vi "Read_MemBank.vi"(8 "error in":errorcluster, 10 "Device":T1, 11 "NNPC_Paths":T2) -> (0 "error out":errorcluster, 3 "NNPC_MemBank_and_Params":T3 {"PreProc_Options"."Dataset_Stats"."stds"."R" format="%#_3g"; "PreProc_Options"."Dataset_Stats"."stds"."G" format="%#_3g"; "PreProc_Options"."Dataset_Stats"."stds"."B" format="%#_3g"; "PreProc_Options"."Dataset_Stats"."means"."R" format="%#_3g"; "PreProc_Options"."Dataset_Stats"."means"."G" format="%#_3g"; "PreProc_Options"."Dataset_Stats"."means"."B" format="%#_3g"; "PreProc_Options"."Interpolation Type" items=["Zero Order", "Bi-Linear", "Quadratic", "Cubic Spline"]; "Evaluation_Results"."Pixel_Range"."Min" format="%#_5g"})   [LabVIEW 2020]
uses:
  Controls/NNPC_MemBank_and_Params.ctl
  <vilib>/Ngene/DeepLTK Anomaly Detection Addon/Toolkit/API/Controls/MemBank_and_Norm_Variants.ctl
  <vilib>/Ngene/DeepLTK Anomaly Detection Addon/Toolkit/API/Controls/NNPC_PreProcessing_Options.ctl
  <vilib>/Ngene/Deep Learning Toolkit/Toolkit/NN_Data/API/NN_Dims(C,H,W).ctl
  <vilib>/Ngene/DeepLTK Anomaly Detection Addon/Toolkit/API/Controls/Crop_CFG.ctl
  <vilib>/Ngene/DeepLTK Anomaly Detection Addon/Toolkit/API/Controls/NNPC_DS_Stats.ctl
  <vilib>/Ngene/DeepLTK Anomaly Detection Addon/Toolkit/API/Controls/Image_Stats_RGB.ctl
  <vilib>/Ngene/DeepLTK Anomaly Detection Addon/Toolkit/API/Controls/NNPC_Evaluation_Results.ctl
  <vilib>/Ngene/DeepLTK Anomaly Detection Addon/Toolkit/API/Controls/NN_Paths.ctl
  <vilib>/Ngene/Deep Learning Toolkit/Toolkit/NN_Network/Controls/NN_Device.ctl
  <vilib>/Ngene/DeepLTK Anomaly Detection Addon/Toolkit/API/Controls/NNPC_Setup.ctl
  <vilib>/Ngene/Deep Learning Toolkit/Toolkit/NN_Network/Controls/NN_Save_Before_Destroy_Options.ctl
  <vilib>/Ngene/CuLab - GPU Accelerated Toolkit/Toolkit/Low_Level/Tensor_Classes/T_Children/T2D/T2D_Children/T2D_SGL/Create_Push.vi
  <vilib>/Ngene/CuLab - GPU Accelerated Toolkit/Toolkit/Low_Level/Tensor_Classes/T_Children/T1D/T1D_Children/T1D_SGL/Create_Push.vi
  <vilib>/Ngene/DeepLTK Anomaly Detection Addon/Toolkit/DeepLTK_Anomaly_Detection_Addon.lvlib
  <vilib>/Ngene/Deep Learning Toolkit/Toolkit/Deep_Learning_Toolkit_by_Ngene.lvlib
  <vilib>/Ngene/CuLab - GPU Accelerated Toolkit/Toolkit/CuLab.lvlib
  <vilib>/Ngene/CuLab - GPU Accelerated Toolkit/Toolkit/Low_Level/Tensor_Classes/T_Children/T1D/T1D_Children/T1D_SGL/T1D_SGL.lvclass
  <vilib>/Ngene/CuLab - GPU Accelerated Toolkit/Toolkit/Low_Level/Tensor_Classes/T_Children/T2D/T2D_Children/T2D_SGL/T2D_SGL.lvclass
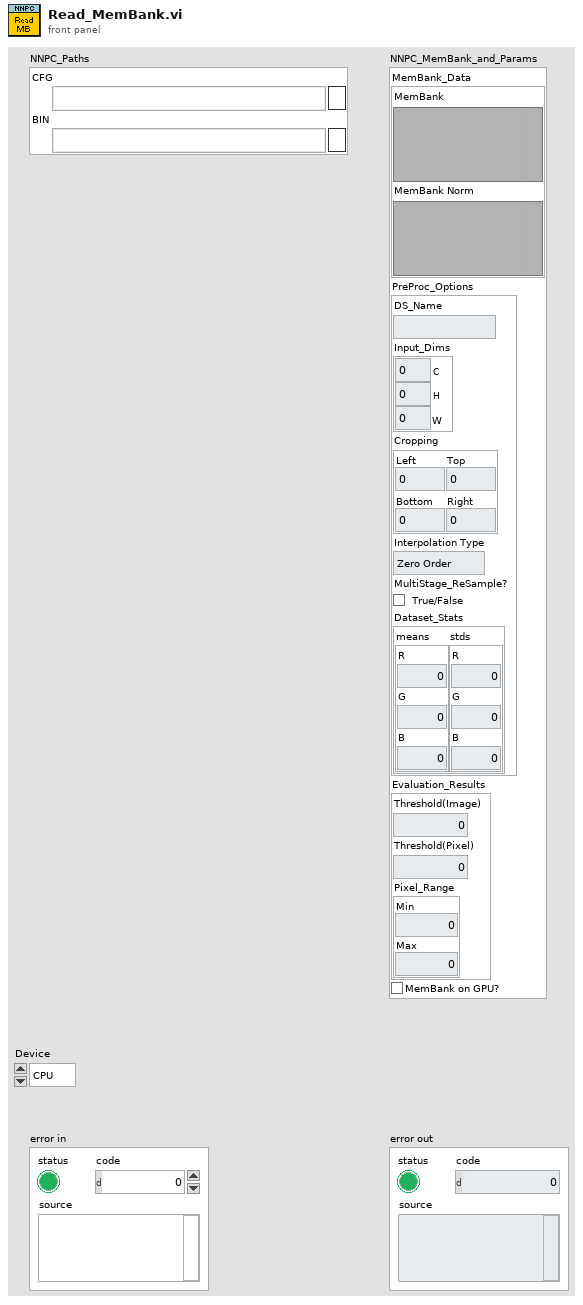
[diagram p1: front panel]
types:
  T1 = typedef "Deep_Learning_Toolkit_by_Ngene.lvlib/NN_Device.ctl" = enum16{"CPU", "GPU"}
  T2 = typedef "DeepLTK_Anomaly_Detection_Addon.lvlib/NN_Paths.ctl" = cluster{"CFG":path, "BIN":path}
  T3 = typedef "NNPC_MemBank_and_Params.ctl" = cluster{"MemBank_Data":T4, "PreProc_Options":T5, "Evaluation_Results":T10, "MemBank on GPU?":bool}
  T4 = typedef "DeepLTK_Anomaly_Detection_Addon.lvlib/MemBank_and_Norm_Variants.ctl" = cluster{"MemBank":variant, "MemBank Norm":variant}
  T5 = typedef "DeepLTK_Anomaly_Detection_Addon.lvlib/NNPC_PreProcessing_Options.ctl" = cluster{"DS_Name":string, "Input_Dims":T6, "Cropping":T7, "Interpolation Type":u32, "MultiStage_ReSample?":bool, "Dataset_Stats":T8}
  T6 = typedef "Deep_Learning_Toolkit_by_Ngene.lvlib/NN_Dims(C,H,W).ctl" = cluster{"C":i32, "H":i32, "W":i32}
  T7 = typedef "DeepLTK_Anomaly_Detection_Addon.lvlib/Crop_CFG.ctl" = cluster{"Left":sgl, "Top":sgl, "Right":sgl, "Bottom":sgl}
  T8 = typedef "DeepLTK_Anomaly_Detection_Addon.lvlib/NNPC_DS_Stats.ctl" = cluster{"means":T9, "stds":T9}
  T9 = typedef "DeepLTK_Anomaly_Detection_Addon.lvlib/Image_Stats_RGB.ctl" = cluster{"R":sgl, "G":sgl, "B":sgl}
  T10 = typedef "DeepLTK_Anomaly_Detection_Addon.lvlib/NNPC_Evaluation_Results.ctl" = cluster{"Threshold(Image)":sgl, "Threshold(Pixel)":sgl, "Pixel_Range":cluster{"Min":sgl, "Max":sgl}}
  T11 = typedef "DeepLTK_Anomaly_Detection_Addon.lvlib/NNPC_Setup.ctl" = cluster{"Input_Dims":T6, "mBatch":i32, "Device":T1, "GPU Id":i32}
  T12 = typedef "Deep_Learning_Toolkit_by_Ngene.lvlib/NN_Save_Before_Destroy_Options.ctl" = cluster{"CFG?":bool, "Weights?":bool, "Render?":bool}
  T13 = typedef "DeepLTK_Anomaly_Detection_Addon.lvlib/NNPC_Instance.ctl" = cluster{"Name":string, "NN":T14, "MemBank_Data":T4}
  T14 = typedef "Deep_Learning_Toolkit_by_Ngene.lvlib/NN.ctl" = cluster{"Name":string, "No of Layers":i32, "mBatch":i32, "Layers":T15[], "Dimty":T16, "Dims_In":T6, "Dims_Out":T6, "Working_Dir":path, "Train?":bool, "Train_Params":T17, "LR_Update_Policy":T20, "Session Data":T22, "Ground_truth":T23, "NNg_hdls":T24, "NN_Device":T1, "GPU Id":i32, "Labels":string[], "Loss_Type":T25, "Loss_Cfg_Prms":variant, "NNG_WS":T26, "DryRun?":bool}
  T15 = typedef "Deep_Learning_Toolkit_by_Ngene.lvlib/NN_Layer_ref.ctl" = refnum<file>
  T16 = typedef "Deep_Learning_Toolkit_by_Ngene.lvlib/NN_In_Out_Dim-ty.ctl" = enum8{"In1D_Out1D", "In3D_Out1D", "In3D_Out3D", "In3D_OutBBox"}
  T17 = typedef "Deep_Learning_Toolkit_by_Ngene.lvlib/NN_Train_Params.ctl" = cluster{"Optimizer":T18, "Beta_1":sgl, "Beta_2":sgl, "Weight Decay(L1)":sgl, "Weight Decay(L2)":sgl, "Data_Sampling":T19}
  T18 = typedef "Deep_Learning_Toolkit_by_Ngene.lvlib/NN_Train_Optimizer.ctl" = enum16{"SGD", "Adam", "Adagrad", "Adadelta", "RMSProp", "Nesterov"}
  T19 = typedef "Deep_Learning_Toolkit_by_Ngene.lvlib/NN_Train_Data_Sampling.ctl" = enum16{"Random", "Sequential"}
  T20 = typedef "Deep_Learning_Toolkit_by_Ngene.lvlib/NN_LR_Policy_Cfg.ctl" = cluster{"Policy_Type":T21, "LR0":dbl, "k":sgl, "WarmUp_Policy":enum16{"Step", "Ramp"}, "WarmUp_Iter":i32, "WarmUp_Ratio":sgl}
  T21 = typedef "Deep_Learning_Toolkit_by_Ngene.lvlib/NN_LR_Policy_Type.ctl" = enum16{"Manual", "Step", "Exp", "1/t"}
  T22 = typedef "Deep_Learning_Toolkit_by_Ngene.lvlib/NN_Train_Session_Data.ctl" = cluster{"Epochs":sgl, "Tot_Iter":i32, "LR":sgl, "LR_iter":i32}
  T23 = typedef "Deep_Learning_Toolkit_by_Ngene.lvlib/NN_Ground_truth.ctl" = cluster{"Y":variant}
  T24 = typedef "Deep_Learning_Toolkit_by_Ngene.lvlib/nng_cuda_handles.ctl" = cluster{"cudnn":u64, "cublas":u64, "stream":u64, "curand":u64}
  T25 = typedef "Deep_Learning_Toolkit_by_Ngene.lvlib/NN_Loss_Type.ctl" = enum16{"None", "MSE", "CrossEntropy", "YOLO_v2", "YOLO_v4"}
  T26 = typedef "Deep_Learning_Toolkit_by_Ngene.lvlib/NNG_WS.ctl" = cluster{"NNG_WS_Mem":T27, "Max_WS_Size":i64}
  T27 = typedef "Deep_Learning_Toolkit_by_Ngene.lvlib/NNg_WS_Mem_DVR.ctl" = refnum<data-value>
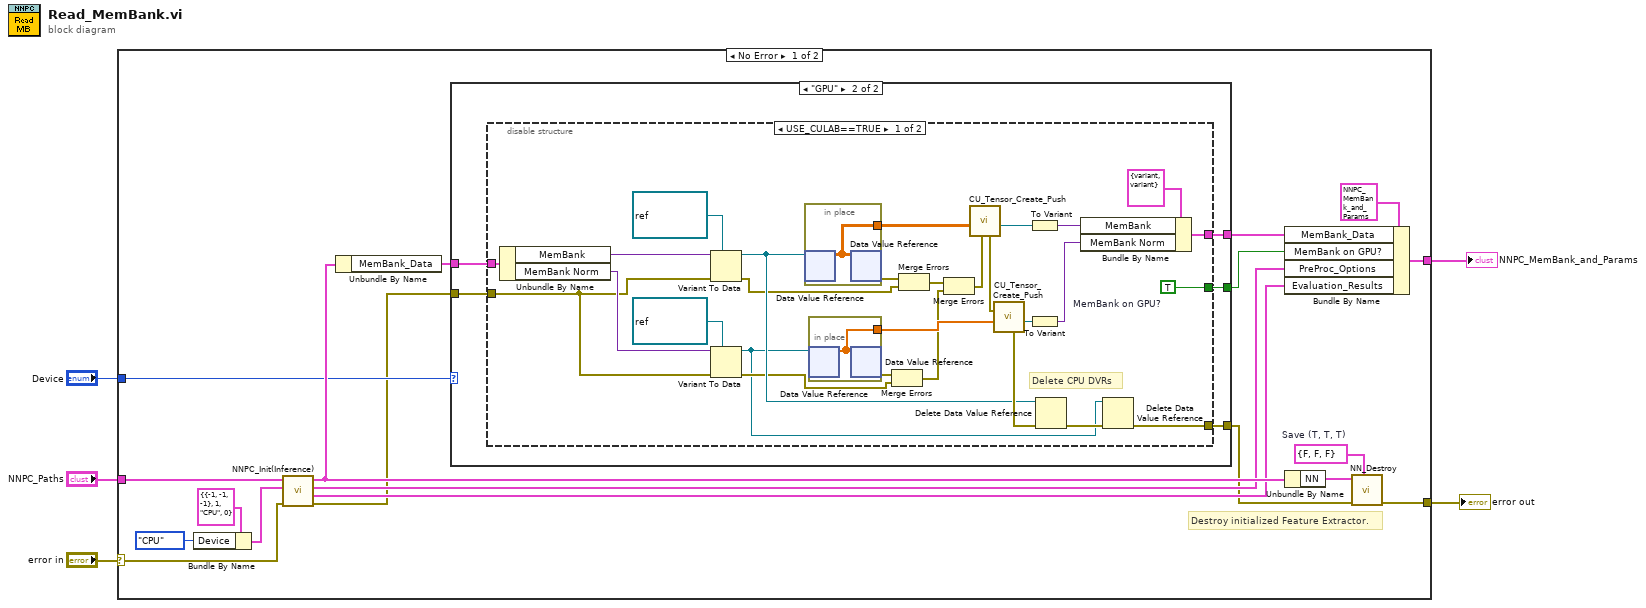
[diagram p0: block diagram]
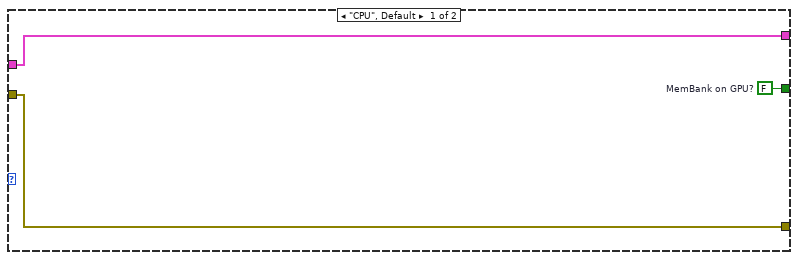
[diagram p2: hidden frame]
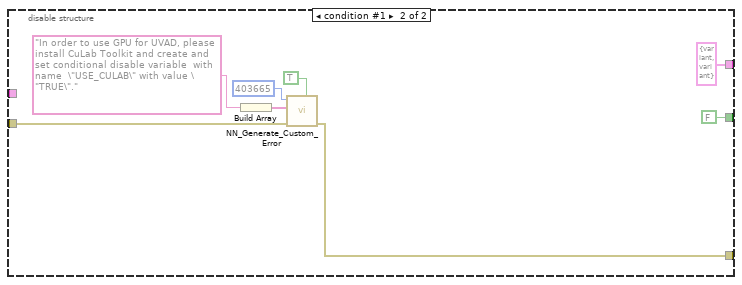
[diagram p3: hidden frame]
diagram:
  n1 = case shown="No Error" "error in" {
    selector: "error in" -> [w24 w71]
    tunnel: [w23 w71] -> w4
    tunnel: [w19 _] -> w3
    tunnel: "NNPC_Paths" -> [w15 _]
    tunnel: "Device" -> [w12 _]
    frame No Error {
      w22 = T12 {"CFG?"=FALSE, "Weights?"=FALSE, "Render?"=FALSE}  # Save (T, T, T)
      # "Destroy initialized Feature Extractor."
      n2 = Bundle By Name(cluster=T11 {"Input_Dims"={"C"=-1, "H"=-1, "W"=-1}, "mBatch"=1, "Device"=enum."CPU", "GPU Id"=0} ("NNPC_Setup"), "Device"=NN_Device."CPU") -> (w13:T11)
      n3 = call <vilib>:"NNPC_Init(Inference).vi"("error in"=w24, "NNPC_Setup"=w13, "NNPC_Paths"=w15) -> ("error out"=w9:errorcluster, "Evaluation_Results"=w18:T10, "PreProc_Options"=w17:T5, "NNPC_out"=w20:T13)  [unwired: 4 in, 1 out]
      n4 = Unbundle By Name(w20) -> ("MemBank_Data"=w11:T4)
      n5 = case shown="\"GPU\"" w12 {
        tunnel: w11 -> [w27 w32]
        tunnel: w9 -> [w26 w31]
        tunnel: [w27 w30] -> w8
        tunnel: [w26 w29] -> w7
        tunnel: [w25 w28] -> w6
        frame "CPU", Default {
          w25 = FALSE  # MemBank on GPU?
        }
        frame "GPU" {
          n6 = disable-structure shown="USE_CULAB==TRUE" {
            disable-tunnel: w32 -> [w60 _]
            disable-tunnel: w31 -> [w50 w66]
            disable-tunnel: [w53 T4 {"MemBank"=variant, "MemBank Norm"=variant} ("MemBank_Data")] -> w30
            disable-tunnel: [w34 w65] -> w29
            disable-tunnel: [w33 FALSE ("MemBank on GPU?")] -> w28
            frame condition #0 (active) {
              w33 = TRUE  # MemBank on GPU?
              # "Delete CPU DVRs"
              n7 = Unbundle By Name(w60) -> ("MemBank"=w58:variant, "MemBank Norm"=w51:variant)
              n8 = Variant To Data(error in=w50, type=refnum<data-value> refnum ("MemBank DVR"), Variant=w58) -> (data=w41:refnum<data-value>, error out=w37:errorcluster)
              n9 = Variant To Data(error in=w50, type=refnum<data-value> refnum ("data value reference"), Variant=w51) -> (data=w35:refnum<data-value>, error out=w39:errorcluster)
              n10 = in-place {
                in-place-border: [w62] -> w57
                n11 = in-place-dvr #1(w41) -> (w62:sgl[][])  [unwired: 1 out]
                n12 = in-place-dvr #1(w62) -> (w46:errorcluster)  [unwired: 1 out]
              }
              n13 = in-place {
                in-place-border: [w61] -> w48
                n14 = in-place-dvr #2(w35) -> (w61:sgl[])  [unwired: 1 out]
                n15 = in-place-dvr #2(w61) -> (w45:errorcluster)  [unwired: 1 out]
              }
              n16 = Merge Errors(w45, w39) -> (w40:errorcluster)
              n17 = Merge Errors(w46, w37) -> (w38:errorcluster)
              n18 = Merge Errors(w38, w40) -> (w47:errorcluster)
              n19 = call-poly <vilib>:"CU_Tensor_Create_Push.vi"("error in (no error)"=w47, "CPU_Data_2D_SGL"=w57) -> ("T2D_SGL out"=w55:refnum<class "T2D_SGL.lvclass">, "error out"=w44:errorcluster)  [unwired: 8 in]
              n20 = call-poly <vilib>:"CU_Tensor_Create_Push.vi"("error in (no error)"=w44, "CPU_Data_1D_SGL"=w48) -> ("T1D_SGL out"=w49:refnum<class "T1D_SGL.lvclass">, "error out"=w42:errorcluster)  [unwired: 8 in]
              n21 = To Variant(anything=w55) -> (Variant=w54:variant)
              n22 = To Variant(anything=w49) -> (Variant=w43:variant)
              n23 = Delete Data Value Reference(data value reference=w41, error in=w42) -> (error out=w36:errorcluster)  [unwired: 1 out]
              n24 = Bundle By Name(cluster=T4 {"MemBank"=variant, "MemBank Norm"=variant} ("MemBank_Data"), "MemBank"=w54, "MemBank Norm"=w43) -> (w53:T4)
              n25 = Delete Data Value Reference(data value reference=w35, error in=w36) -> (error out=w34:errorcluster)  [unwired: 1 out]
            }
            frame condition #1 {
              n26 = Build Array("In order to use GPU for UVAD, please install CuLab Toolkit and create and set conditional disable variable  with name  \"USE_CULAB\" with value \"TRUE\"." ("Message")) -> (w69:string[])
              n27 = call <vilib>:"NN_Generate_Custom_Error.vi"("show call chain? (TRUE)"=TRUE ("show call chain? (False)"), "error in (no error)"=w66, "Message"=w69, "Error_code"=403665) -> ("error out"=w65:errorcluster)  [unwired: 7 in]
            }
          }
        }
      }
      n28 = Bundle By Name(cluster=T3 {"MemBank_Data"={"MemBank"=variant, "MemBank Norm"=variant}, "PreProc_Options"={"DS_Name"="", "Input_Dims"={"C"=-1, "H"=-1, "W"=-1}, "Cropping"={"Left"=0.0, "Top"=0.0, "Right"=1.0, "Bottom"=1.0}, "Interpolation Type"=1, "MultiStage_ReSample?"=FALSE, "Dataset_Stats"={"means"={"R"=0.5385, "G"=0.5348, "B"=0.551}, "stds"={"R"=0.3673, "G"=0.3673, "B"=0.3505}}}, "Evaluation_Results"={"Threshold(Image)"=0.0, "Threshold(Pixel)"=0.0, "Pixel_Range"={"Min"=0.0, "Max"=0.0}}, "MemBank on GPU?"=FALSE}, "MemBank_Data"=w8, "MemBank on GPU?"=w6, "PreProc_Options"=w17, "Evaluation_Results"=w18) -> (w19:T3)
      n29 = Unbundle By Name(w20) -> ("NN"=w21:T14)
      n30 = call <vilib>:"NN_Destroy.vi"("Save (T, T, T)"=w22, "error in (no error)"=w7, "NN in"=w21) -> ("error out"=w23:errorcluster)  [unwired: 7 in, 1 out]
    }
    frame Error {
    }
  }
  "error out" <- w4
  "NNPC_MemBank_and_Params" <- w3
